vi "mean_strain__b41b222be2.vi"(8 "Iteration":dbl, 10 "current":dbl[](array[numeric]), 11 "real strain":dbl[](array[numeric])) -> (0 "mean current(A)":dbl, 1 "min strain (-)":dbl, 2 "mean strain (-)":dbl, 3 "max strain (-)":dbl, 4 "min current":dbl, 5 "max current":dbl)   [LabVIEW 2023]
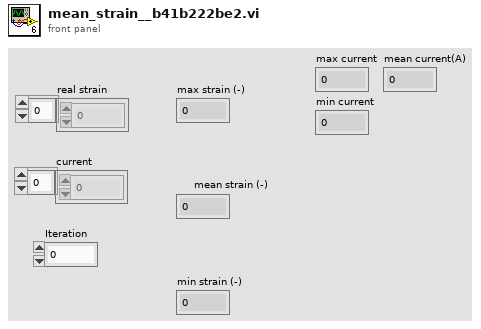
[diagram p1: front panel]
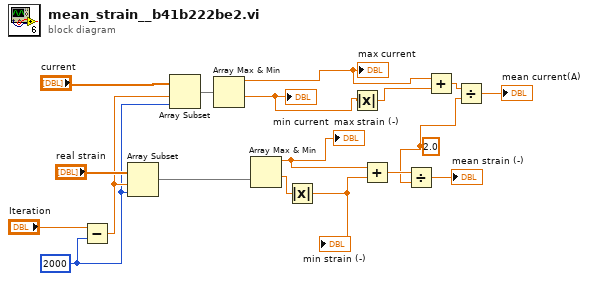
[diagram p0: block diagram]
diagram:
  w8 = 2000
  w2 = 2.0 ("y")
  n1 = Subtract(x="Iteration", y=w8) -> (x-y=w9:dbl)
  n2 = Array Subset(array="real strain", index=w9, length=w8) -> (w12:dbl[])
  n3 = Array Subset(array="current", index=w9, length=w8) -> (w7:dbl[])
  n4 = Array Max & Min(array=w7) -> (max value=w6:dbl, min value=w4:dbl)  [unwired: 2 out]
  "max current" <- w6
  "min current" <- w4
  n5 = Array Max & Min(array=w12) -> (max value=w16:dbl, min value=w15:dbl)  [unwired: 2 out]
  "max strain (-)" <- w16
  n6 = Absolute Value(x=w15) -> (abs(x)=w14:dbl)
  "min strain (-)" <- w14
  n7 = Absolute Value(x=w4) -> (abs(x)=w5:dbl)
  n8 = Add(x=w16, y=w14) -> (x+y=w17:dbl)
  n9 = Divide(x=w17, y=w2) -> (x/y=→"mean strain (-)":dbl)
  n10 = Add(x=w6, y=w5) -> (x+y=w3:dbl)
  n11 = Divide(x=w3, y=w2) -> (x/y=→"mean current(A)":dbl)
